vi "GOOP_GetClassDynamicVIs.vi"(0 "LvClassIn":refnum<vi>, 5 "error in":errorcluster) -> (9 "IsMustOverride":bool[](array[boolean]), 11 "IsAPropertyDefinitionVI":bool[](array[boolean]), 13 "ConnectorPaneHeight":i32[](array[numeric]), 14 "LvClassOut":refnum<vi>, 15 "ClassName":string, 16 "VINames(without Prefix)":string[](array[string]), 17 "ViPaths":path[](array[path]), 18 "Scope":T1(array[ring]), 19 "error out":errorcluster)   [LabVIEW 2020]
panel:
  # "0 or -1 means Full Icon height\n1 is only one connector terminal height\n  and the header is then removed."
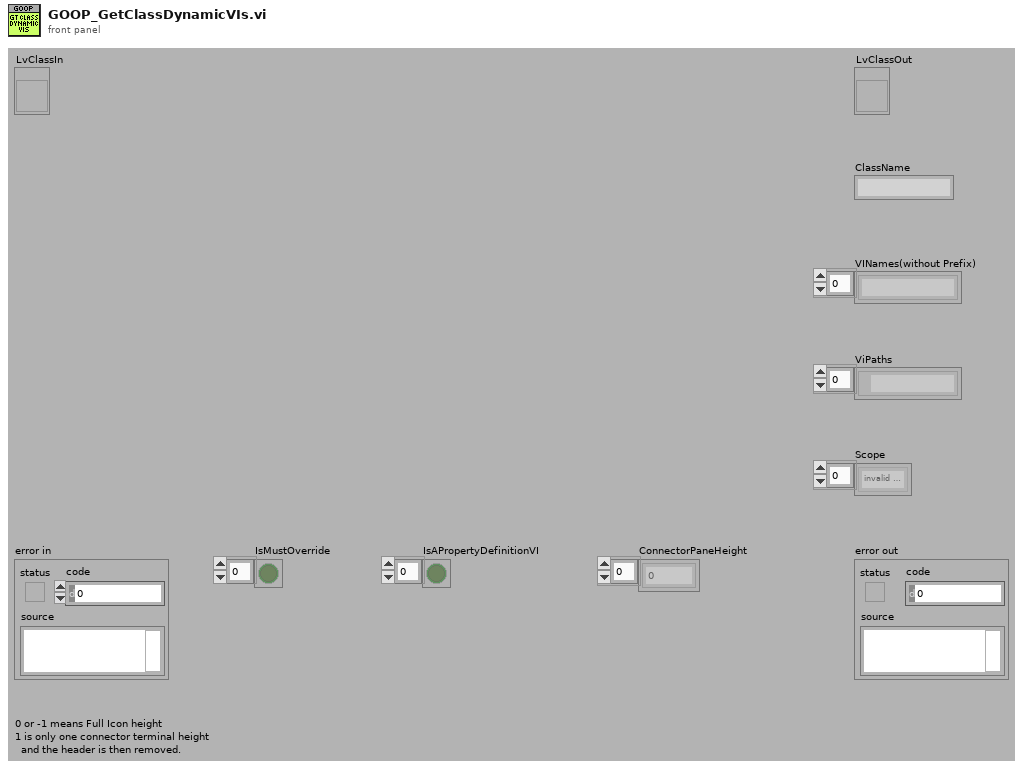
[diagram p1: front panel]
types:
  T1 = enum32{"invalid scope", "public", "private", "protected", "community"}[]
  T2 = enum16{"Invalid Wire Rule", "Required", "Recommended", "Optional", "Dynamic Dispatch"}
  T3 = enum32{"invalid scope", "public", "private", "protected", "community"}
  T4 = enum16{"Invalid Wire Rule", "Required", "Recommended", "Optional", "Dynamic Dispatch"}[]
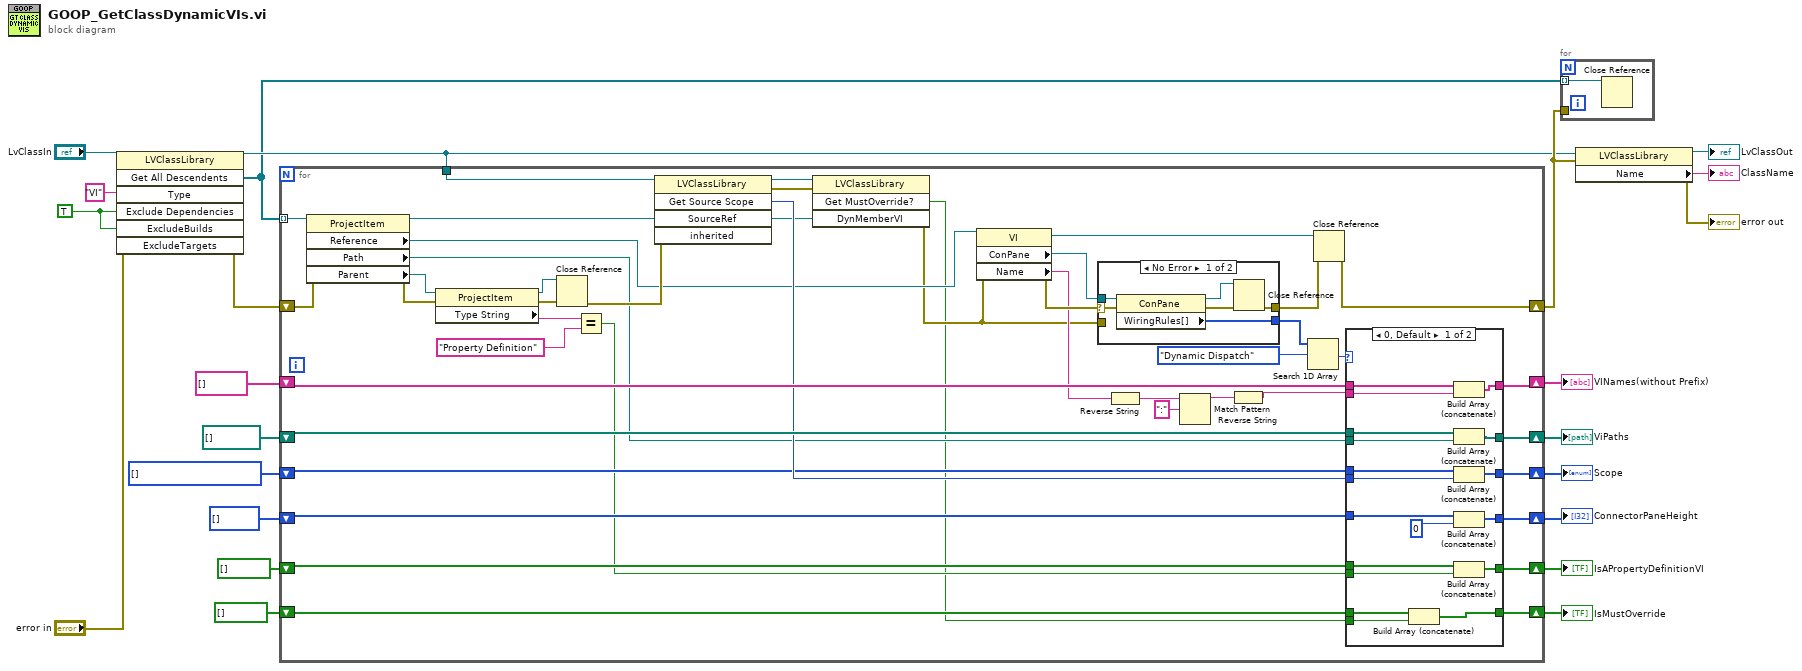
[diagram p0: block diagram]
diagram:
  w11 = TRUE ("ExcludeDependencies")
  w13 = T1 [] items=["invalid scope", "public", "private", "protected", "community"]
  n1 = invoke class="LVClassLibrary" method="Get All Descendents"(reference="LvClassIn", error in="error in", "Type"="VI", "Exclude Dependencies"=w11, "ExcludeBuilds"=w11) -> (reference out=w9:refnum<vi>, error out=w5:errorcluster, "All Descendents"=w8:refnum<vi>[])  [unwired: 2 in, 4 out]
  n2 = for {
    tunnel: w8 -> [w67] mode=indexing
    shift-right: [w59] -> w10
    shift-left: w5 -> [w66]
    shift-right: [w60] -> w23
    shift-left: string[] [] ("Array 2") -> [w61]
    shift-right: [w57] -> w14
    shift-left: path[] [] -> [w56]
    shift-right: [w53] -> w12
    shift-left: w13 -> [w50]
    tunnel: w9 -> [w52]
    shift-right: [w45] -> w7
    shift-left: i32[] [] ("ConnectorPaneHeight") -> [w46]
    shift-right: [w35] -> w3
    shift-left: bool[] [] -> [w34]
    shift-right: [w26] -> w1
    shift-left: bool[] [] -> [w25]
    n3 = property class="ProjectItem"(reference=w67, error in=w66) -> (reference out=w27:refnum<vi>, error out=w39:errorcluster, "Reference"=w31:refnum<vi>, "Path"=w32:path, "Parent"=w42:refnum<vi>)
    n4 = property class="ProjectItem"(reference=w42, error in=w39) -> (reference out=w40:refnum<vi>, error out=w41:errorcluster, "Type String"=w37:string)
    n5 = Close Reference(reference=w40, error in (no error)=w41) -> (error out=w38:errorcluster)
    n6 = Equal?(x=w37, y="Property Definition" ("Type String 2")) -> (x = y?=w33:bool)
    n7 = invoke class="LVClassLibrary" method="Get Source Scope"(reference=w52, error in=w38, "SourceRef"=w27) -> (reference out=w30:refnum<vi>, error out=w29:errorcluster, "GetSourceScope"=w51:T3)  [unwired: 2 in, 2 out]
    n8 = invoke class="LVClassLibrary" method="Get MustOverride?"(reference=w30, error in=w29, "DynMemberVI"=w27) -> (error out=w28:errorcluster, "GetMustOverride"=w24:bool)  [unwired: 1 in, 2 out]
    n9 = property class="VI"(reference=w31, error in=w28) -> (reference out=w43:refnum<vi>, error out=w58:errorcluster, "ConPane"=w44:refnum<vi>, "Name"=w55:string)
    n10 = case shown="No Error" w58 {
      selector: w58 -> [w69 _]
      tunnel: w44 -> [w73 _]
      tunnel: [w72 _] -> w65
      tunnel: [w70 w74] -> w63
      tunnel: w28 -> [_ w74]
      frame No Error {
        n11 = property class="ConPane"(reference=w73, error in=w69) -> (reference out=w68:refnum<vi>, error out=w71:errorcluster, "WiringRules[]"=w72:T4)
        n12 = Close Reference(reference=w68, error in (no error)=w71) -> (error out=w70:errorcluster)
      }
      frame Error {
      }
    }
    n13 = Reverse String(1:w55) -> (0:w49:string)
    n14 = Match Pattern(string=w49, regular expression=":") -> (before substring=w48:string)  [unwired: 1 in, 3 out]
    n15 = Reverse String(1:w48) -> (0:w47:string)
    n16 = Search 1D Array(1D array=w65, element=T2."Dynamic Dispatch") -> (index of element=w62:i32)  [unwired: 1 in]
    n17 = Close Reference(reference=w43, error in (no error)=w63) -> (error out=w59:errorcluster)
    n18 = case shown="0, Default" w62 {
      tunnel: w61 -> [w92 w98]
      tunnel: [w91 w98] -> w60
      tunnel: w47 -> [w90 _]
      tunnel: [w87 w97] -> w57
      tunnel: w56 -> [w89 w97]
      tunnel: w32 -> [w88 _]
      tunnel: [w86 w96] -> w53
      tunnel: w51 -> [w85 _]
      tunnel: w50 -> [w84 w96]
      tunnel: [w82 w95] -> w45
      tunnel: w46 -> [w83 w95]
      tunnel: [w80 w94] -> w35
      tunnel: w34 -> [w79 w94]
      tunnel: w33 -> [w78 _]
      tunnel: [w76 w93] -> w26
      tunnel: w25 -> [w77 w93]
      tunnel: w24 -> [w75 _]
      frame 0, Default {
        # "We need to examine the Connector Pane"
        n19 = Build Array (concatenate)(w77, w75) -> (w76:bool[])
        n20 = Build Array (concatenate)(w92, w90) -> (w91:string[])
        n21 = Build Array (concatenate)(w89, w88) -> (w87:path[])
        n22 = Build Array (concatenate)(w84, w85) -> (w86:T1)
        n23 = Build Array (concatenate)(w83, 0 ("Numeric")) -> (w82:i32[])
        n24 = Build Array (concatenate)(w79, w78) -> (w80:bool[])
      }
      frame -1 {
      }
    }
  }
  "VINames(without Prefix)" <- w23
  "ViPaths" <- w14
  "Scope" <- w12
  "ConnectorPaneHeight" <- w7
  "IsAPropertyDefinitionVI" <- w3
  "IsMustOverride" <- w1
  n25 = for {
    tunnel: w10 -> [_]
    tunnel: w8 -> [w99] mode=indexing
    n26 = Close Reference(reference=w99) -> ()  [unwired: 1 in, 1 out]
  }
  n27 = property class="LVClassLibrary"(reference=w9, error in=w10) -> (reference out=→"LvClassOut":refnum<vi>, error out=→"error out":errorcluster, "Name"=→"ClassName":string)
